vi "PhotonMultiTargetPNPResult_unpack.vi"(9 "StartByte":i32, 11 "RawData":u8[](array[numeric])) -> (1 "NextByte":i32, 3 "MultiTargetPNP_Result":T1={"PhotonPNPResult"={"IsPresent"=FALSE, "bestReprojErr"=0.0, "altReprojErr"=0.0, "ambiguity"=0.0, "Best"={"TRANSLATION3D"={"X"=0.0, "Y"=0.0, "Z"=0.0}, "ROTATION3D"={"Q_quaternion"={"R"=1.0, "V"=[0.0, 0.0, 0.0]}}, "XF"=FALSE}, "Alt"={"TRANSLATION3D"={"X"=0.0, "Y"=0.0, "Z"=0.0}, "ROTATION3D"={"Q_quaternion"={"R"=1.0, "V"=[0.0, 0.0, 0.0]}}, "XF"=FALSE}}, "FiducialIDsUsed"=[]} {"PhotonPNPResult"."Alt"."TRANSLATION3D"."Z" format="%14.3f"; "PhotonPNPResult"."Alt"."TRANSLATION3D"."Y" format="%14.3f"; "PhotonPNPResult"."Alt"."TRANSLATION3D"."X" format="%14.3f"; "PhotonPNPResult"."Best"."TRANSLATION3D"."Z" format="%14.3f"; "PhotonPNPResult"."Best"."TRANSLATION3D"."Y" format="%14.3f"; "PhotonPNPResult"."Best"."TRANSLATION3D"."X" format="%14.3f"})   [LabVIEW 2019, in "PhotonVisionLib.lvlib"]
doc: "Internal function to parse the data for MultiTargetPNPResult\n\nInputs:\n - RawData -- Byte array containing the data to parse.\n - StartingByte - Index into RawData to start parsing. Beginning of data is index 0.\n\nOutputs:\n - MultiTargetPNPResult -- Parsed result cluster.\n - NextByte -- Index to byte following ths data in RawData."
uses:
  PhotonVisionLib.lvlib
  <vilib>/Rock Robotics/WPI/ThirdParty/JAS_Junk/TrajLib/TypeDef/TRANSLATION3D.ctl
  <vilib>/Rock Robotics/WPI/ThirdParty/JAS_Junk/TrajLib/Trajectory_Library.lvlib
  <vilib>/Rock Robotics/WPI/ThirdParty/JAS_Junk/TrajLib/TypeDef/QUATERNION.ctl
  <vilib>/Rock Robotics/WPI/ThirdParty/JAS_Junk/TrajLib/TypeDef/ROTATION3D.ctl
  <vilib>/Rock Robotics/WPI/ThirdParty/JAS_Junk/TrajLib/TypeDef/TRANSFORM3D.ctl
  TypeDef/PhotonPNPResultType.ctl
  TypeDef/PhotonMultiTargetPNPResultType.ctl
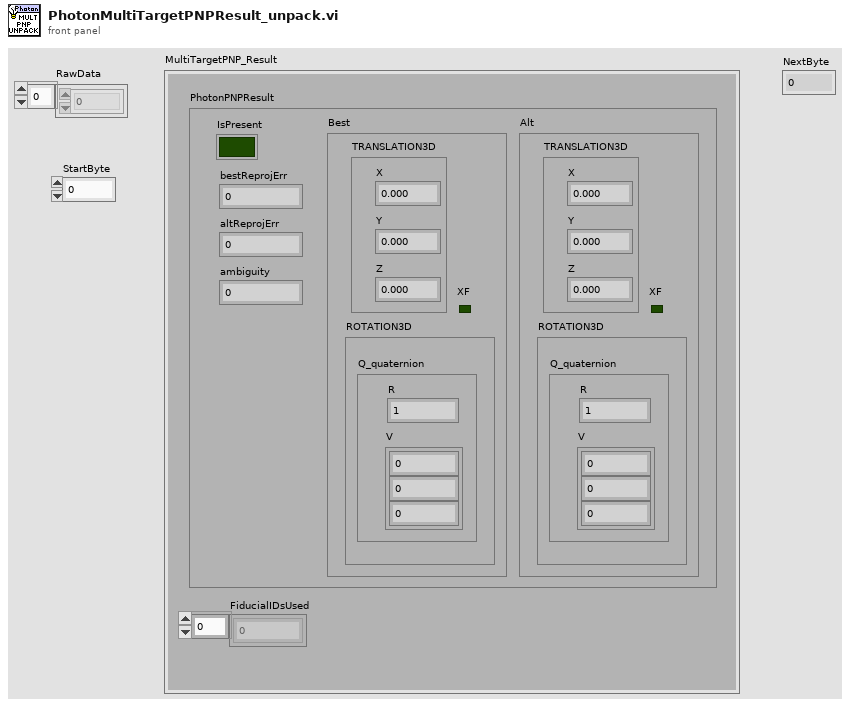
[diagram p1: front panel]
types:
  T1 = typedef "PhotonVisionLib.lvlib/PhotonMultiTargetPNPResultType.ctl" = cluster{"PhotonPNPResult":T2, "FiducialIDsUsed":i16[]}
  T2 = typedef "PhotonVisionLib.lvlib/PhotonPNPResultType.ctl" = cluster{"IsPresent":bool, "bestReprojErr":dbl, "altReprojErr":dbl, "ambiguity":dbl, "Best":T3, "Alt":T3}
  T3 = typedef "Trajectory_Library.lvlib/TRANSFORM3D.ctl" = cluster{"TRANSLATION3D":T4, "ROTATION3D":T5, "XF":bool}
  T4 = typedef "Trajectory_Library.lvlib/TRANSLATION3D.ctl" = cluster{"X":dbl, "Y":dbl, "Z":dbl}
  T5 = typedef "Trajectory_Library.lvlib/ROTATION3D.ctl" = cluster{"Q_quaternion":T6}
  T6 = typedef "Trajectory_Library.lvlib/QUATERNION.ctl" = cluster{"R":dbl, "V":dbl[]}
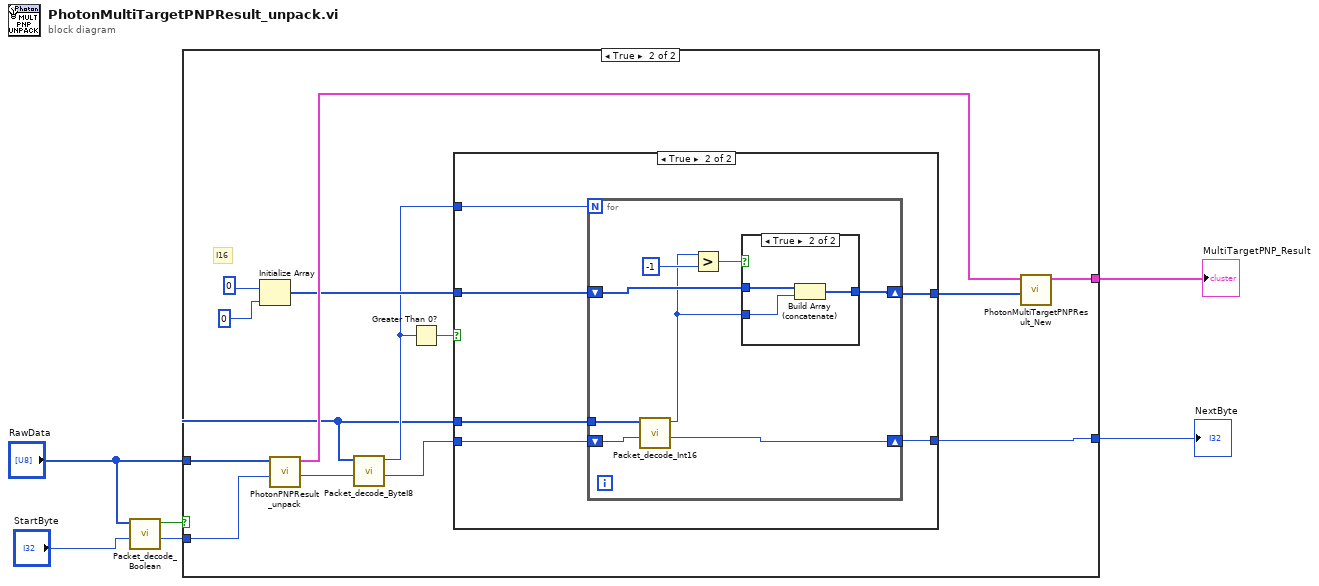
[diagram p0: block diagram]
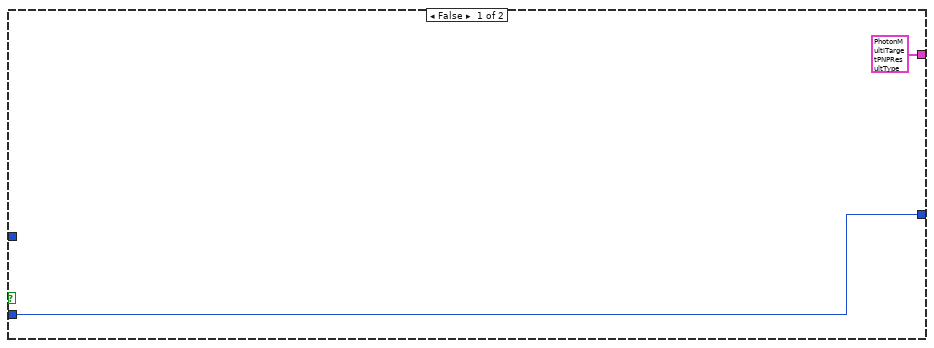
[diagram p2: hidden frame]
diagram:
  n1 = call "Packet_decode_Boolean.vi"("StartByte"="StartByte", "RawData"="RawData") -> ("NextByte"=w1:i32, "Boolean_Value"=w2:bool)  [unwired: 8 in]
  n2 = case shown="True" w2 {
    tunnel: [T1 {"PhotonPNPResult"={"IsPresent"=FALSE, "bestReprojErr"=0.0, "altReprojErr"=0.0, "ambiguity"=0.0, "Best"={"TRANSLATION3D"={"X"=0.0, "Y"=0.0, "Z"=0.0}, "ROTATION3D"={"Q_quaternion"={"R"=1.0, "V"=[0.0, 0.0, 0.0]}}, "XF"=FALSE}, "Alt"={"TRANSLATION3D"={"X"=0.0, "Y"=0.0, "Z"=0.0}, "ROTATION3D"={"Q_quaternion"={"R"=1.0, "V"=[0.0, 0.0, 0.0]}}, "XF"=FALSE}}, "FiducialIDsUsed"=[]} ("MultiTargetPNPResult") w21] -> w6
    tunnel: [w8 w19] -> w5
    tunnel: "RawData" -> [_ w10]
    tunnel: w1 -> [w8 w9]
    frame False {
    }
    frame True {
      # "I16"
      n3 = Initialize Array(i16 0, 0 ("dimension size")) -> (w16:i16[])
      n4 = call "PhotonPNPResult_unpack.vi"("StartByte"=w9, "RawData"=w10) -> ("NextByte"=w14:i32, "PNP_Result"=w20:T2)  [unwired: 8 in]
      n5 = call "Packet_decode_ByteI8.vi"("StartByte"=w14, "RawData"=w10) -> ("NextByte"=w13:i32, "Int8_Value"=w11:i8)  [unwired: 8 in]
      n6 = Greater Than 0?(x=w11) -> (x > 0?=w12:bool)
      n7 = case shown="True" w12 {
        tunnel: [w22 w29] -> w19
        tunnel: w16 -> [w23 w28]
        tunnel: [w23 w27] -> w15
        tunnel: w10 -> [_ w26]
        tunnel: w11 -> [_ w25]
        tunnel: w13 -> [w22 w24]
        frame False {
        }
        frame True {
          n8 = for {
            N: w25 -> [_]
            tunnel: w26 -> [w37]
            shift-right: [w35] -> w29
            shift-left: w24 -> [w36]
            shift-right: [w30] -> w27
            shift-left: w28 -> [w32]
            n9 = call "Packet_decode_Int16.vi"("StartByte"=w36, "RawData"=w37) -> ("NextByte"=w35:i32, "Int16_Value"=w31:i16)  [unwired: 8 in]
            n10 = Greater?(x=w31, y=i16 -1) -> (0:w33:bool)
            n11 = case shown="True" w33 {
              tunnel: w32 -> [w38 w41]
              tunnel: w31 -> [_ w40]
              tunnel: [w38 w39] -> w30
              frame False {
              }
              frame True {
                n12 = Build Array (concatenate)(w41, w40) -> (w39:i16[])
              }
            }
          }
        }
      }
      n13 = call "PhotonMultiTargetPNPResult_New.vi"("FiducialIDsUsed"=w15, "PhotonPNPResult"=w20) -> ("MultiTargetPNPResult"=w21:T1)  [unwired: 9 in]
    }
  }
  "MultiTargetPNP_Result" <- w6
  "NextByte" <- w5
